vi "MQTT Data Stream - Decode Varint.vi"(8 "error in (no error)":errorcluster, 9 "timeout ms (1000)":i32, 11 "TCP Network Connection in":refnum<k5>) -> (0 "error out":errorcluster, 1 "Size (bytes)":i32, 2 "Numeric":u32, 3 "TCP Network Connection out":refnum<k5>, 5 "RAW data":string)   [LabVIEW 2019, in "KoRE-MQTT.lvlib"]
doc: "Copyright (c) 2025 KoRElibs.com\nSPDX-License-Identifier: EUPL-1.2\n\nThis VI is licensed under the European Union Public License (EUPL) Version 1.2. You may use this VI unmodified in proprietary works. If you distribute a modified version of this file, the modified file must be released under the EUPL-1.2. Full license: https://joinup.ec.europa.eu/asset/eupl/eupl/1.2/"
uses:
  KoRE-MQTT.lvlib
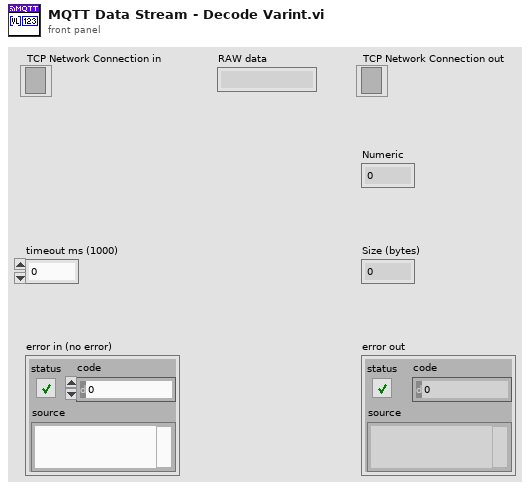
[diagram p1: front panel]
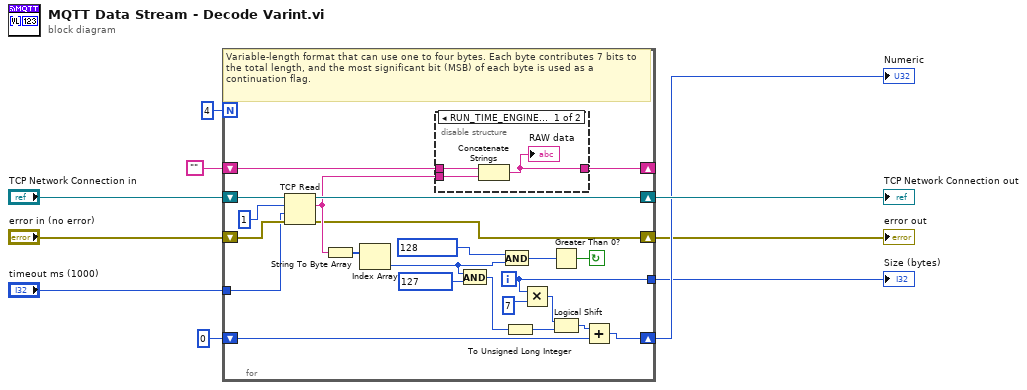
[diagram p0: block diagram]
diagram:
  n1 = for {
    N: 4 -> [_]
    shift-right: [w27] -> w6
    shift-left: u32 0 -> [w26]
    tunnel: [w22] -> w4
    shift-right: [w18] -> w7
    shift-left: "TCP Network Connection in" -> [w17]
    shift-right: [w12] -> _
    shift-left: "" -> [w16]
    shift-right: [w13] -> w5
    shift-left: "error in (no error)" -> [w14]
    tunnel: "timeout ms (1000)" -> [w11]
    i -> [w22]
    stop <- w30 continue-if-true
    # "Variable-length format that can use one to four bytes. Each byte contributes 7 bits to the total length, and the most significant bit (MSB) of each byte is used as a continuation flag."
    n2 = TCP Read(connection ID=w17, bytes to read=1, error in (no error)=w14, 9:w11) -> (connection ID out=w18:refnum<k5>, data out=w15:string, error out=w13:errorcluster)  [unwired: 1 in]
    n3 = String To Byte Array(string=w15) -> (unsigned byte array=w20:u8[])
    n4 = Index Array(array=w20) -> (element=w19:u8)  [unwired: 1 in]
    n5 = disable-structure shown="RUN_TIME_ENGINE==False" {
      disable-tunnel: w16 -> [w36 w37]
      disable-tunnel: w15 -> [w35 _]
      disable-tunnel: [w34 w37] -> w12
      frame condition #0 (active) {
        n6 = Concatenate Strings(w36, w35) -> (w34:string)
        "RAW data" <- w34
      }
      frame condition #1 {
      }
    }
    n7 = And(x=w19, y=u8 127) -> (x .and. y?=w29:u8)
    n8 = And(x=u8 128, y=w19) -> (x .and. y?=w31:u8)
    n9 = To Unsigned Long Integer(number=w29) -> (unsigned 32bit integer=w25:u32)
    n10 = Multiply(x=w22, y=7) -> (x*y=w28:i32)
    n11 = Greater Than 0?(x=w31) -> (x > 0?=w30:bool)
    n12 = Logical Shift(y=w28, x=w25) -> (x << y=w24:u32)
    n13 = Add(x=w24, y=w26) -> (x+y=w27:u32)
  }
  "TCP Network Connection out" <- w7
  "Numeric" <- w6
  "error out" <- w5
  "Size (bytes)" <- w4
